vi "test progress legacy cancel.vi"(8 "error in (no error)":errorcluster) -> (0 "error out":errorcluster, 3 "body":string)   [LabVIEW 2020, in "MCP Server tests.lvlib"]
doc: "Legacy cancellation (MCP 2025-06-18 and older). A legacy streamed tools/call of fake_tool_progress runs on a raw TCP connection; after its first progress event, notifications/cancelled with its id is POSTed on a second connection. That is answered with HTTP 202 at once (Process HTTP Request.vi is not blocked by the streamed call), Report Progress.vi returns cancelled? TRUE, the tool stops early, and the stream ends without a result."
uses:
  MCP Server tests.lvlib
  cf8b1df6-8b76-4ce7-be9c-a9ee1466f89a.vi
  <vilib>/JDP Science/JSONtext/Next JSON Value.vi
  <vilib>/JDP Science/JSONtext/String Subset.vi
  <vilib>/JDP Science/JSONtext/Parsing/Advance past next JSON Value (inlined COPY).vi
  <vilib>/JDP Science/JSONtext/Parsing/Advance past whitespace.vi
  <vilib>/JDP Science/JSONtext/Parsing/Advance past String.vi
  <vilib>/JDP Science/JSONtext/Parsing/Advance past Number.vi
  <vilib>/JDP Science/JSONtext/Parsing/Advance past Line Ending.vi
  <vilib>/JDP Science/JSONtext/Parsing/Parse Full Path or Item Name.vi
  <vilib>/JDP Science/JSONtext/Parsing/Advance past Array.vi
  <vilib>/JDP Science/JSONtext/Parsing/Advance past Object.vi
  <vilib>/JDP Science/JSONtext/support/Error Cluster From Code.vi
  <vilib>/JDP Science/JSONtext/Offset/Find Item Locations by Path.vi
  <vilib>/JDP Science/JSONtext/JSON text to Variant.vi
  <vilib>/JDP Science/JSONtext/LVClass Serializer/JSONtext LVClass Serializer.lvclass
  <vilib>/addons/_JKI Toolkits/Caraya/classes/Test/Test.lvclass
  <vilib>/addons/_JKI Toolkits/Caraya/classes/Assert/Assert.lvclass
  <vilib>/JDP Science/JSONtext/JSONtext.lvlib
panel:
  out "lookup error":errorcluster
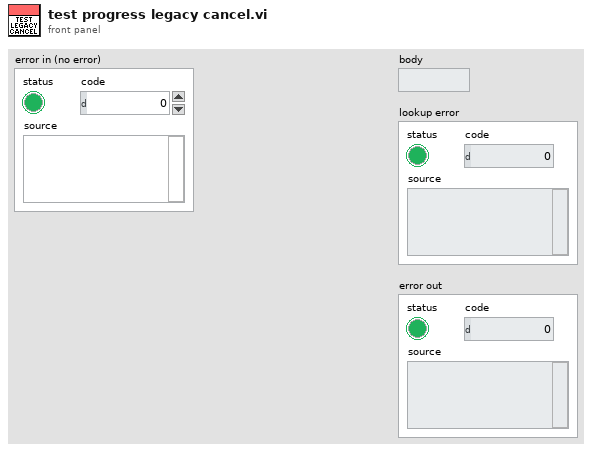
[diagram p1: front panel]
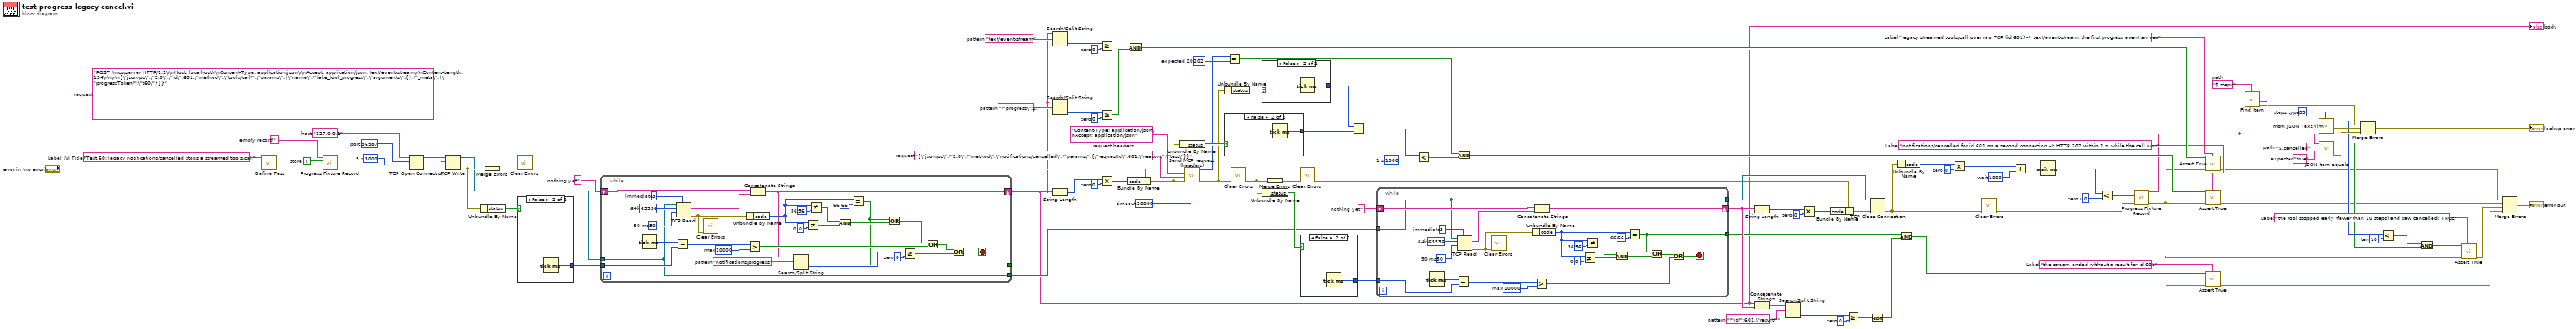
[diagram p0: block diagram]
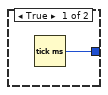
[diagram p2: hidden frame]
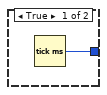
[diagram p3: hidden frame]
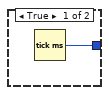
[diagram p4: hidden frame]
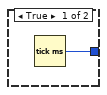
[diagram p5: hidden frame]
diagram:
  w73 = "Content-Type: application/json\nAccept: application/json"  # request headers
  w24 = "the stream ended without a result for id 601"  # Label
  w8 = "the tool stopped early (fewer than 10 steps) and saw cancelled? TRUE"  # Label
  w26 = "notifications/cancelled for id 601 on a second connection -> HTTP 202 within 1 s, while the call runs"  # Label
  w28 = "legacy streamed tools/call over raw TCP (id 601) -> text/event-stream, the first progress event arrives"  # Label
  w45 = 0  # zero
  w49 = "\"id\":601,\"result\""  # pattern
  w18 = "true"  # expected
  w19 = "$.cancelled"  # path
  w13 = 10  # ten
  w59 = u32 1000  # 1 s
  w67 = 202  # expected 202
  w79 = 0  # zero
  w85 = "\"progress\":1,"  # pattern
  w81 = 0  # zero
  w86 = "text/event-stream"  # pattern
  w21 = 99  # steps type
  w23 = "$.steps"  # path
  w32 = u32 0  # zero u
  w35 = 1000  # wait
  w37 = 0  # zero
  w51 = 0  # zero
  w56 = ""  # nothing yet
  w71 = 20000  # timeout
  w72 = "{\"jsonrpc\":\"2.0\",\"method\":\"notifications/cancelled\",\"params\":{\"requestId\":601,\"reason\":\"test\"}}"  # request
  w83 = 0  # zero
  w87 = ""  # nothing yet
  w94 = "POST /mcp/server HTTP/1.1\r\nHost: localhost\r\nContent-Type: application/json\r\nAccept: application/json, text/event-stream\r\nContent-Length: 134\r\n\r\n{\"jsonrpc\":\"2.0\",\"id\":601,\"method\":\"tools/call\",\"params\":{\"name\":\"fake_tool_progress\",\"arguments\":{},\"_meta\":{\"progressToken\":\"t60\"}}}"  # request
  w97 = 5000  # 5 s
  w98 = u16 36987  # port
  w99 = "127.0.0.1"  # host
  w101 = TRUE  # store
  w102 = ""  # empty record
  w104 = "Test 60: legacy notifications/cancelled stops a streamed tools/call"  # Label (VI Title)
  n1 = call <vilib>:"Define Test.vi"("error in (no error)"="error in (no error)", "Label (VI Title)"=w104) -> ("error out"=w100:errorcluster)  [unwired: 8 in, 1 out]
  n2 = call "Progress Fixture Record.vi"("error in"=w100, "set?"=w101, "record in"=w102) -> ("error out"=w96:errorcluster)  [unwired: 7 in, 1 out]
  n3 = TCP Open Connection(address=w99, remote port or service name=w98, timeout ms (60000)=w97, error in (no error)=w96) -> (connection ID=w95:refnum<k5>, error out=w93:errorcluster)  [unwired: 1 in]
  n4 = TCP Write(connection ID=w95, data in=w94, error in (no error)=w93) -> (connection ID out=w89:refnum<k5>, error out=w92:errorcluster)  [unwired: 1 in, 1 out]
  n5 = Unbundle By Name(w92) -> ("status"=w91:bool)
  n6 = Merge Errors(w92) -> (w90:errorcluster)
  n7 = call <vilib>:"Clear Errors.vi"("error in (no error)"=w90) -> ("error out"=w77:errorcluster)  [unwired: 5 in, 1 out]
  n8 = case shown="False" w91 {
    tunnel: [w105 w106] -> w88
    frame True {
      n9 = Tick Count (ms)() -> (millisecond timer value=w105:u32)
    }
    frame False {
      n10 = Tick Count (ms)() -> (millisecond timer value=w106:u32)
    }
  }
  n11 = while {
    tunnel: w89 -> [w108]
    tunnel: w88 -> [w130]
    shift-right: [w110] -> w3
    shift-left: w87 -> [w109]
    tunnel: [w108] -> w58
    tunnel: [w107] -> _
    stop <- w111 stop-if-true
    w117 = 0  # zero
    w121 = "notifications/progress"  # pattern
    w126 = u32 10000  # max
    w122 = 0  # 0
    w124 = 56  # 56
    w125 = 66  # 66
    w132 = u16 3  # immediate
    w133 = 50  # 50 ms
    w134 = 65536  # 64k
    n12 = Tick Count (ms)() -> (millisecond timer value=w131:u32)
    n13 = Subtract(x=w131, y=w130) -> (x-y=w127:u32)
    n14 = TCP Read(connection ID=w108, bytes to read=w134, 7:w132, 9:w133) -> (data out=w128:string, error out=w129:errorcluster)  [unwired: 1 in, 1 out]
    n15 = call <vilib>:"Clear Errors.vi"("error in (no error)"=w129) -> ()  [unwired: 5 in, 2 out]
    n16 = Unbundle By Name(w129) -> ("code"=w123:i32)
    n17 = Greater?(x=w127, y=w126) -> (0:w114:bool)
    n18 = Concatenate Strings(w109, w128) -> (w110:string)
    n19 = Search/Split String(string=w110, search string/char (-)=w121) -> (offset of match=w118:i32)  [unwired: 1 in, 2 out]
    n20 = Not Equal?(x=w123, y=w122) -> (x != y?=w119:bool)
    n21 = Not Equal?(x=w123, y=w124) -> (x != y?=w120:bool)
    n22 = And(x=w120, y=w119) -> (x .and. y?=w116:bool)
    n23 = Equal?(x=w123, y=w125) -> (x = y?=w107:bool)
    n24 = Or(x=w107, y=w116) -> (x .or. y?=w115:bool)
    n25 = Greater Or Equal?(x=w118, y=w117) -> (x >= y?=w112:bool)
    n26 = Or(x=w115, y=w114) -> (x .or. y?=w113:bool)
    n27 = Or(x=w113, y=w112) -> (x .or. y?=w111:bool)
  }
  "body" <- w3
  n28 = Search/Split String(string=w3, search string/char (-)=w86) -> (offset of match=w82:i32)  [unwired: 1 in, 2 out]
  n29 = Search/Split String(string=w3, search string/char (-)=w85) -> (offset of match=w80:i32)  [unwired: 1 in, 2 out]
  n30 = String Length(string=w3) -> (length=w84:i32)
  n31 = Greater Or Equal?(x=w82, y=w81) -> (x >= y?=w76:bool)
  n32 = Greater Or Equal?(x=w80, y=w79) -> (x >= y?=w75:bool)
  n33 = Multiply(x=w84, y=w83) -> (x*y=w78:i32)
  n34 = Bundle By Name(cluster=w77, "code"=w78) -> (w70:errorcluster)
  n35 = And(x=w76, y=w75) -> (x .and. y?=w29:bool)
  n36 = Unbundle By Name(w70) -> ("status"=w74:bool)
  n37 = call "Send MCP request (headers).vi"("timeout (10000)"=w71, "error in (no error)"=w70, "request"=w72, "request headers"=w73) -> ("error out"=w69:errorcluster, "status code"=w68:i32)  [unwired: 4 in, 2 out]
  n38 = Unbundle By Name(w69) -> ("status"=w66:bool)
  n39 = case shown="False" w74 {
    tunnel: [w135 w136] -> w63
    frame True {
      n40 = Tick Count (ms)() -> (millisecond timer value=w135:u32)
    }
    frame False {
      n41 = Tick Count (ms)() -> (millisecond timer value=w136:u32)
    }
  }
  n42 = Equal?(x=w68, y=w67) -> (x = y?=w55:bool)
  n43 = call <vilib>:"Clear Errors.vi"("error in (no error)"=w69) -> ("error out"=w65:errorcluster)  [unwired: 5 in, 1 out]
  n44 = case shown="False" w66 {
    tunnel: [w137 w138] -> w64
    frame True {
      n45 = Tick Count (ms)() -> (millisecond timer value=w137:u32)
    }
    frame False {
      n46 = Tick Count (ms)() -> (millisecond timer value=w138:u32)
    }
  }
  n47 = Unbundle By Name(w65) -> ("status"=w62:bool)
  n48 = Merge Errors(w65) -> (w61:errorcluster)
  n49 = call <vilib>:"Clear Errors.vi"("error in (no error)"=w61) -> ("error out"=w47:errorcluster)  [unwired: 5 in, 1 out]
  n50 = case shown="False" w62 {
    tunnel: [w139 w140] -> w57
    frame True {
      n51 = Tick Count (ms)() -> (millisecond timer value=w139:u32)
    }
    frame False {
      n52 = Tick Count (ms)() -> (millisecond timer value=w140:u32)
    }
  }
  n53 = Subtract(x=w64, y=w63) -> (x-y=w60:u32)
  n54 = while {
    tunnel: w58 -> [w142]
    tunnel: w57 -> [w159]
    shift-right: [w144] -> w53
    shift-left: w56 -> [w143]
    tunnel: [w142] -> w44
    tunnel: [w141] -> w40
    stop <- w145 stop-if-true
    w155 = u32 10000  # max
    w151 = 0  # 0
    w153 = 56  # 56
    w154 = 66  # 66
    w161 = u16 3  # immediate
    w162 = 50  # 50 ms
    w163 = 65536  # 64k
    n55 = Tick Count (ms)() -> (millisecond timer value=w160:u32)
    n56 = Subtract(x=w160, y=w159) -> (x-y=w156:u32)
    n57 = TCP Read(connection ID=w142, bytes to read=w163, 7:w161, 9:w162) -> (data out=w157:string, error out=w158:errorcluster)  [unwired: 1 in, 1 out]
    n58 = call <vilib>:"Clear Errors.vi"("error in (no error)"=w158) -> ()  [unwired: 5 in, 2 out]
    n59 = Unbundle By Name(w158) -> ("code"=w152:i32)
    n60 = Greater?(x=w156, y=w155) -> (0:w146:bool)
    n61 = Concatenate Strings(w143, w157) -> (w144:string)
    n62 = Not Equal?(x=w152, y=w151) -> (x != y?=w149:bool)
    n63 = Not Equal?(x=w152, y=w153) -> (x != y?=w150:bool)
    n64 = And(x=w150, y=w149) -> (x .and. y?=w148:bool)
    n65 = Equal?(x=w152, y=w154) -> (x = y?=w141:bool)
    n66 = Or(x=w141, y=w148) -> (x .or. y?=w147:bool)
    n67 = Or(x=w147, y=w146) -> (x .or. y?=w145:bool)
  }
  n68 = Less?(x=w60, y=w59) -> (x < y?=w54:bool)
  n69 = And(x=w55, y=w54) -> (x .and. y?=w27:bool)
  n70 = String Length(string=w53) -> (length=w52:i32)
  n71 = Concatenate Strings(w3, w53) -> (w50:string)
  n72 = Search/Split String(string=w50, search string/char (-)=w49) -> (offset of match=w46:i32)  [unwired: 1 in, 2 out]
  n73 = Multiply(x=w52, y=w51) -> (x*y=w48:i32)
  n74 = Bundle By Name(cluster=w47, "code"=w48) -> (w43:errorcluster)
  n75 = Greater Or Equal?(x=w46, y=w45) -> (x >= y?=w42:bool)
  n76 = Not(x=w42) -> (.not. x?=w39:bool)
  n77 = TCP Close Connection(connection ID=w44, error in (no error)=w43) -> (error out=w41:errorcluster)  [unwired: 1 in, 1 out]
  n78 = Unbundle By Name(w41) -> ("code"=w38:i32)
  n79 = And(x=w40, y=w39) -> (x .and. y?=w25:bool)
  n80 = Multiply(x=w38, y=w37) -> (x*y=w36:i32)
  n81 = call <vilib>:"Clear Errors.vi"("error in (no error)"=w41) -> ("error out"=w30:errorcluster)  [unwired: 5 in, 1 out]
  n82 = Add(x=w36, y=w35) -> (x+y=w34:i32)
  n83 = Wait (ms)(milliseconds to wait=w34) -> (millisecond timer value=w33:u32)
  n84 = Less?(x=w33, y=w32) -> (x < y?=w31:bool)
  n85 = call "Progress Fixture Record.vi"("error in"=w30, "set?"=w31) -> ("error out"=w9:errorcluster, "record out"=w20:string)  [unwired: 8 in]
  n86 = call <vilib>:"Assert True.vi"("Label"=w28, "error in (no error)"=w9, "True?"=w29) -> ("error out"=w7:errorcluster)  [unwired: 7 in, 1 out]
  n87 = call <vilib>:"Assert True.vi"("Label"=w26, "error in (no error)"=w9, "True?"=w27) -> ("error out"=w6:errorcluster)  [unwired: 7 in, 1 out]
  n88 = call <vilib>:"Assert True.vi"("Label"=w24, "error in (no error)"=w9, "True?"=w25) -> ("error out"=w4:errorcluster)  [unwired: 7 in, 1 out]
  n89 = call <vilib>:"Find Item.vi"("$Path or Item Name"=w23, "JSON"=w20) -> ("error out"=w17:errorcluster, "<JSON>"=w22:string)  [unwired: 6 in, 2 out]
  n90 = call "From JSON Text.vim"("Data Type and Default Value"=w21, "JSON"=w22) -> ("error out"=w16:errorcluster, "Data out"=w14:i32)  [unwired: 8 in]
  n91 = call "JSON item equals.vi"("expected"=w18, "path"=w19, "JSON"=w20) -> ("error out"=w15:errorcluster, "equal?"=w11:bool)  [unwired: 6 in, 1 out]
  n92 = Merge Errors(w17, w16, w15) -> (→"lookup error":errorcluster)
  n93 = Less?(x=w14, y=w13) -> (x < y?=w12:bool)
  n94 = And(x=w12, y=w11) -> (x .and. y?=w10:bool)
  n95 = call <vilib>:"Assert True.vi"("Label"=w8, "error in (no error)"=w9, "True?"=w10) -> ("error out"=w5:errorcluster)  [unwired: 7 in, 1 out]
  n96 = Merge Errors(w7, w6, w5, w4) -> (→"error out":errorcluster)
